vi "RFH-convert_folder-r140.vi"(3 "pre-modifier":string="R140-", 5 "Destination Folder":path, 7 "Folder Path":path, 8 "source":string, 9 "Max Frequency (6G)":dbl=6000000000.0, 10 "Min Frequency  (0.3G)":dbl=300000000.0, 11 "Xi":dbl[](array[numeric])) -> (0 "error out":errorcluster, 2 "All Good?":bool, 4 "Last Value":T1)   [LabVIEW 2020, in "RFH-Reflection_File_Handler.lvlib"]
doc: "Converts all R140 Excel files of a folder to the common format on the frequencies Xi, limited to the min and max frequency, saves them and verifies the conversion."
uses:
  RFH-Reflection_File_Handler.lvlib
  RFH-common_data_format.ctl
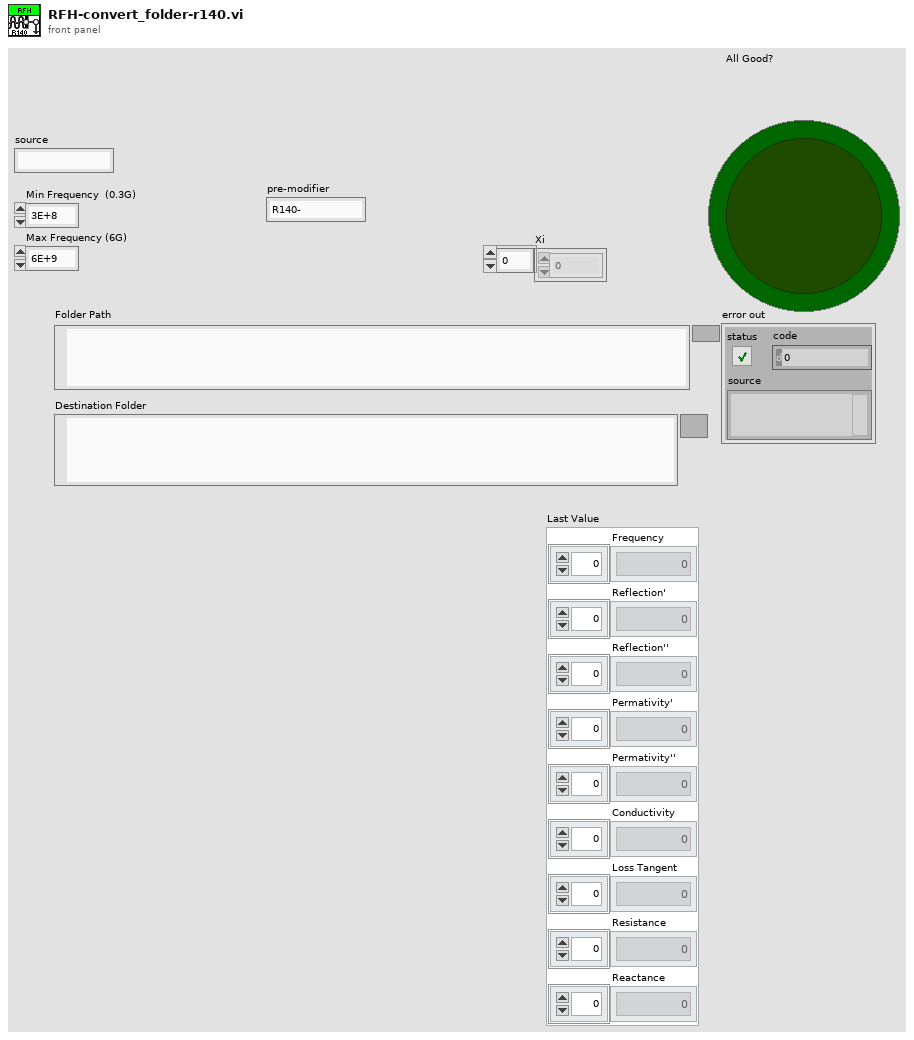
[diagram p1: front panel]
types:
  T1 = typedef "RFH-Reflection_File_Handler.lvlib/RFH-common_data_format.ctl" = cluster{"Frequency":dbl[], "Reflection'":dbl[], "Reflection''":dbl[], "Permativity'":dbl[], "Permativity''":dbl[], "Conductivity":dbl[], "Loss Tangent":dbl[], "Resistance":dbl[], "Reactance":dbl[]}
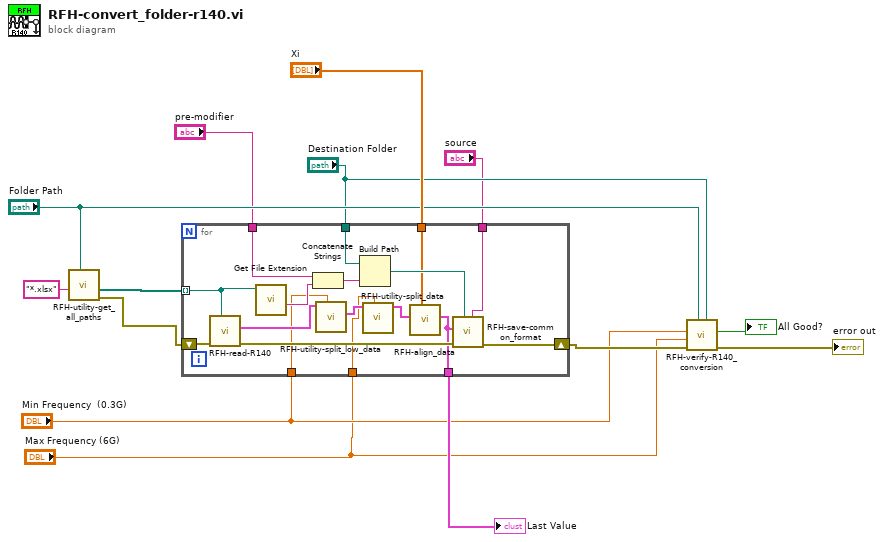
[diagram p0: block diagram]
diagram:
  n1 = call "RFH-utility-get_all_paths.vi"("Folder Path"="Folder Path", "pattern"="*.xlsx") -> ("error out"=w13:errorcluster, "All Files in Dir"=w14:path[])  [unwired: 6 in, 2 out]
  n2 = for {
    tunnel: w14 -> [w31] mode=indexing
    tunnel: "Destination Folder" -> [w28]
    shift-right: [w25] -> w7
    shift-left: w13 -> [w24]
    tunnel: "Xi" -> [w23]
    tunnel: [w22] -> w5
    tunnel: "pre-modifier" -> [w21]
    tunnel: "Min Frequency  (0.3G)" -> [w17]
    tunnel: "Max Frequency (6G)" -> [w16]
    tunnel: "source" -> [w15]
    n3 = call "RFH-read-R140.vi"("file path (dialog if empty)"=w31, "error in (no error)"=w24) -> ("error out"=w26:errorcluster, "Common Format"=w19:T1)  [unwired: 7 in, 1 out]
    n4 = call <vilib>:"Get File Extension.vi"("file"=w31) -> ("filename without extension"=w30:string)  [unwired: 6 in, 4 out]
    n5 = Concatenate Strings(w21, w30) -> (w29:string)
    n6 = call "RFH-utility-split_low_data.vi"("Frequency"=w17, "Common Format"=w19) -> ("After"=w20:T1)  [unwired: 9 in]
    n7 = Build Path(base path=w28, name or relative path=w29) -> (appended path=w27:path)
    n8 = call "RFH-utility-split_data.vi"("Frequency"=w16, "Common Format"=w20) -> ("Before"=w18:T1)  [unwired: 8 in, 1 out]
    n9 = call "RFH-align_data.vi"("Xi"=w23, "Common Format"=w18) -> ("Common Format alligned"=w22:T1)  [unwired: 9 in]
    n10 = call "RFH-save-common_format.vi"("source"=w15, "file path (use dialog)"=w27, "error in (no error)"=w26, "Common Format"=w22) -> ("error out"=w25:errorcluster)  [unwired: 7 in]
  }
  "Last Value" <- w5
  n11 = call "RFH-verify-R140_conversion.vi"("Conversion Folder"="Destination Folder", "Excel File Folder"="Folder Path", "error in (no error)"=w7, "Max Frequency (6G)"="Max Frequency (6G)", "Min Frequency  (0.3G)"="Min Frequency  (0.3G)") -> ("error out"=→"error out":errorcluster, "All Good?"=→"All Good?":bool)  [unwired: 5 in]
